vi "Call.vi"(7 "Actor in":refnum<class "Actor.lvclass">, 8 "Error in":errorcluster, 9 "Parent Stopped":bool, 10 "Safe Stop":bool=TRUE) -> (0 "Error out":errorcluster, 5 "Actor out":refnum<class "Actor.lvclass">)   [LabVIEW 2020, in "jettl.lvlib" / "Stop jettl Msg.lvlib" / "Stop.lvlib"]
uses:
  Stop.lvlib
  Actor/Actor.lvclass
  Stop Msg Input/Stop Msg Input/Stop Msg Input.lvclass/Stop Msg Input.ctl
  Stop Msg/Stop Msg/Stop Msg.lvclass/Stop Msg.ctl
  Init Msg.vi
  Stop Msg/Init Msg.vi
  Stop Msg Input/Init Msg Input.vi
  Stop Msg/Stop Msg/Init Msg.vi
  Stop Msg Input/Stop Msg Input/Init Msg Input.vi
  Stop Msg Input/Stop Msg Input/Stop Msg Input.lvclass
  C:/git/jettl/src/jettl/jettl/Msg Input/Msg Input.lvclass
  Stop Msg/Stop Msg/Stop Msg.lvclass
  C:/git/jettl/src/jettl/jettl/Msg/Msg.lvclass
  Teller/Teller.lvclass
  Stop Msg Output/Stop Msg Output/Stop Msg Output.lvclass
  jettl.lvlib
  Stop Msg Output/Stop Msg Output.lvlib
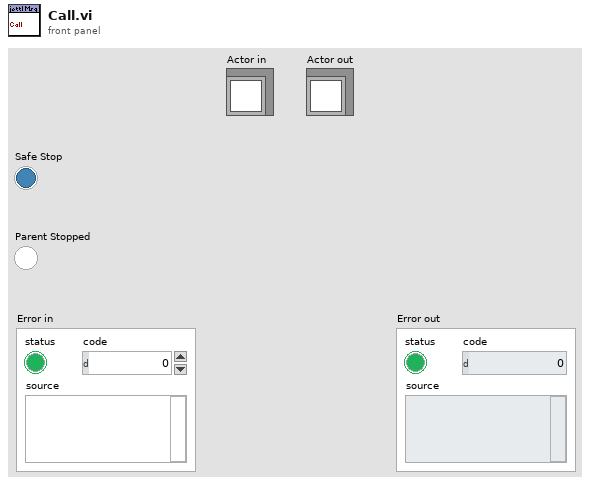
[diagram p1: front panel]
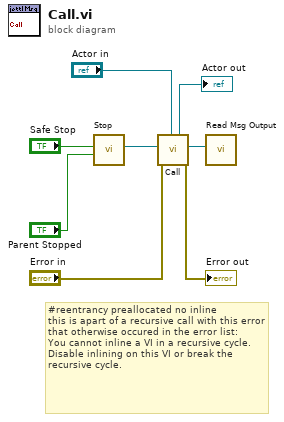
[diagram p0: block diagram]
diagram:
  # "#reentrancy preallocated no inline\nthis is apart of a recursive call with this error that otherwise occured in the error list:\nYou cannot inline a VI in a recursive cycle. Disable inlining on this VI or break the recursive cycle."
  n1 = call-poly "Stop.vi"("Parent Stopped"="Parent Stopped", "Safe Stop"="Safe Stop") -> ("Msg"=w3:refnum<class "Msg.lvclass">)  [unwired: 9 in]
  n2 = call "Call.vi"("Actor in"="Actor in", "Error in"="Error in", "Msg"=w3) -> ("Error out"=→"Error out":errorcluster, "Msg Output"=w4:refnum<class "Msg Output.lvclass">, "Actor out"=→"Actor out":refnum<class "Actor.lvclass">)  [unwired: 6 in]
  n3 = call "Read Msg Output.vi"("Msg Output"=w4) -> ()  [unwired: 11 in]
